vi "Write U8 External Payload.vi"(8 "error in (no error)":errorcluster, 9 "Timeout (ms)":i32, 10 "U8 With Header in":u8[](array[numeric]), 11 "CIF_Iceoryx_PCAP_Universal in":refnum<class "CIF_Iceoryx_PCAP_Universal.lvclass">) -> (0 "error out":errorcluster, 1 "timed out?":bool, 2 "U8 With Header out":u8[](array[numeric]), 3 "CIF_Iceoryx_PCAP_Universal out":refnum<class "CIF_Iceoryx_PCAP_Universal.lvclass">)   [LabVIEW 2021, in "CIF_Iceoryx_PCAP_Universal.lvclass"]
uses:
  CIF_Iceoryx_PCAP_Universal.lvclass
  D:/dev/Packages/CIF_Channels_Core/src/CIFChannels/CIFChannels.lvclass
  CIFChannels/CIFChannels.lvclass/CIFChannels.ctl
  CIF_Iceoryx_PCAP_Universal.lvclass/CIF_Iceoryx_PCAP_Universal.ctl
  <vilib>/CIF Foundation/CIF Utilities/Statistics/I64/Stats_I64_CIF_U.lvclass/Stats_I64_CIF_U.ctl
  006b6af1-e7ad-4c5f-a9a8-941eabcd64fe.vi
  98bb9657-57c0-4b2f-8932-fd51e6c7d0e2.vi
  CIFChannels/Accessors/Read FIFO Backpressure.vi
  <vilib>/CIF Foundation/CIF Utilities/Statistics/I64/X1 minus X0.vi
  <vilib>/CIF Foundation/CIF Utilities/Time/System Time/Get System Time.vi
  <vilib>/CIF Foundation/CIF Iceoryx/SubVIs/Get Path.vi
  <vilib>/CIF Foundation/CIF Iceoryx/SubVIs/Convert Error.vi
  <vilib>/CIF Foundation/CIF Iceoryx/Refnum/CIF Publisher from Refnum.vi
  <vilib>/CIF Foundation/CIF Utilities/Statistics/I64/X1 minus X0.vi/dfabcf33-0dbc-4041-80a5-3dc0c86d2989.vi
  <vilib>/CIF Foundation/CIF Utilities/Statistics/I64/X1 minus X0.vi/dfabcf33-0dbc-4041-80a5-3dc0c86d2989.vi/9eb60a9a-770f-4d2d-8b3f-8465c267ecc9.vi
  <vilib>/CIF Foundation/CIF Iceoryx/PubSub/CIF pcap/Get CIF Subscriber Count.vi
  <vilib>/CIF Foundation/CIF Iceoryx/SubVIs/Convert Error Core.vi
  CIFChannels/CIFChannels.lvclass
  <vilib>/CIF Foundation/CIF Iceoryx/Iceoryx.lvlib
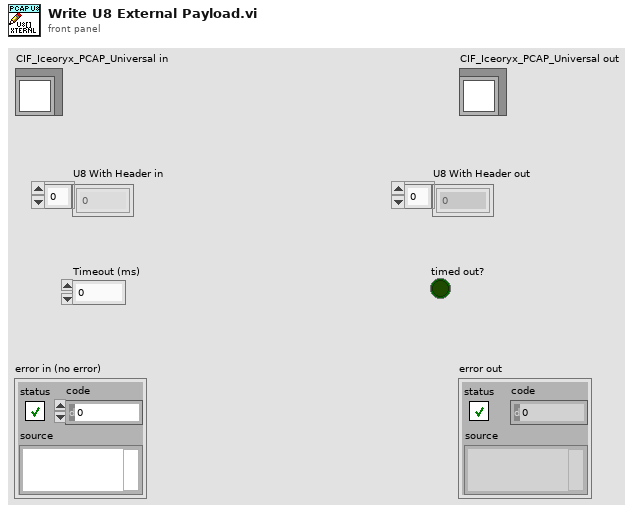
[diagram p1: front panel]
types:
  T1 = typedef "Iceoryx.lvlib/CIF Publisher Refnum.ctl" = cluster{"refnum":u64, "CIF Pub":enum8{"cifpub"}}
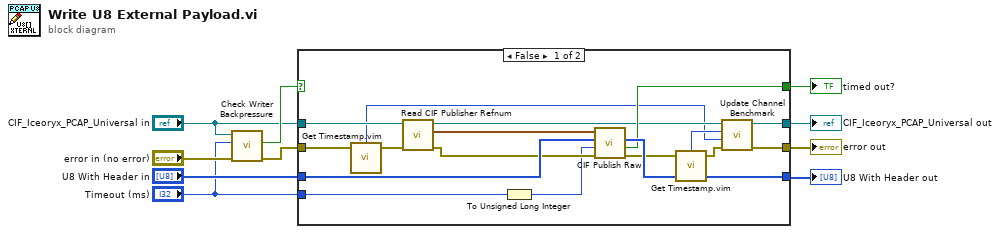
[diagram p0: block diagram]
diagram:
  n1 = call "Check Writer Backpressure.vi"("error in (no error)"="error in (no error)", "Timeout (ms)"="Timeout (ms)", "CIF_CIPC_Chn in"="CIF_Iceoryx_PCAP_Universal in") -> ("error out"=w10:errorcluster, "timed out?"=w9:bool)  [unwired: 7 in]
  n2 = case shown="False" w9 {
    selector: w9 -> [_ w29]
    tunnel: [w27 w31] -> w3
    tunnel: [w26 w28] -> w5
    tunnel: "U8 With Header in" -> [w25 w30]
    tunnel: "CIF_Iceoryx_PCAP_Universal in" -> [w23 w28]
    tunnel: w10 -> [w22 w31]
    tunnel: [w24 w30] -> w2
    tunnel: "Timeout (ms)" -> [w21 _]
    tunnel: [w20 w29] -> w4
    frame False {
      n3 = call "Get Timestamp.vim"("Anything in"=w22) -> ("Time (ns)"=w11:i64, "Anything out"=w12:errorcluster)  [unwired: 2 in]
      n4 = call "Read CIF Publisher Refnum.vi"("error in (no error)"=w12, "CIF_Iceoryx_PCAP_Universal in"=w23) -> ("error out"=w15:errorcluster, "CIF Publisher Refnum"=w14:T1, "CIF_Iceoryx_PCAP_Universal out"=w16:refnum<class "CIF_Iceoryx_PCAP_Universal.lvclass">)  [unwired: 7 in]
      n5 = To Unsigned Long Integer(number=w21) -> (unsigned 32bit integer=w13:u32)
      n6 = call <vilib>:"CIF Publish Raw.vi"("error in (no error)"=w15, "Timoeut ms"=w13, "Data In"=w25, "Publisher Reference"=w14) -> ("error out"=w17:errorcluster, "Timeout"=w20:bool, "Data Out"=w24:u8[])  [unwired: 4 in, 1 out]
      n7 = call "Get Timestamp.vim"("Anything in"=w17) -> ("Time (ns)"=w19:i64, "Anything out"=w18:errorcluster)  [unwired: 2 in]
      n8 = call "Update Channel Benchmark.vi"("error in (no error)"=w18, "X0"=w11, "X1"=w19, "CIFChannels in"=w16) -> ("error out"=w27:errorcluster, "CIFChannels out"=w26:refnum<class "CIF_Iceoryx_PCAP_Universal.lvclass">)  [unwired: 6 in]
    }
    frame True {
    }
  }
  "error out" <- w3
  "CIF_Iceoryx_PCAP_Universal out" <- w5
  "timed out?" <- w4
  "U8 With Header out" <- w2
